vi "Connect FSV.vi"(8 "error in (no error)":errorcluster caption="에러 입력(에러 없음)", 10 "VISA resource name":refnum<visa-resource-name>, 11 "Instrument Manager 입력":refnum<class "Instrument Manager.lvclass">) -> (0 "error out":errorcluster caption="에러 출력", 3 "Instrument Manager 출력":refnum<class "Instrument Manager.lvclass">)   [LabVIEW 2023, in "Instrument Manager.lvclass"]
uses:
  Instrument Manager.lvclass
  Instrument Manager.lvclass/Instrument Manager.ctl
  Module/Spectrum Analyzer/Class/FSV-40N/FSV-40N.lvclass
  C:/Users/HCT-3320/Documents/Instrument Manger/Module/Spectrum Analyzer/Class/FSV-40N/FSV-40N.lvclass
  C:/Users/HCT-3320/Documents/Instrument Manger/Module/Spectrum Analyzer/Interface_Spectrum/Interface_Spectrum.lvclass
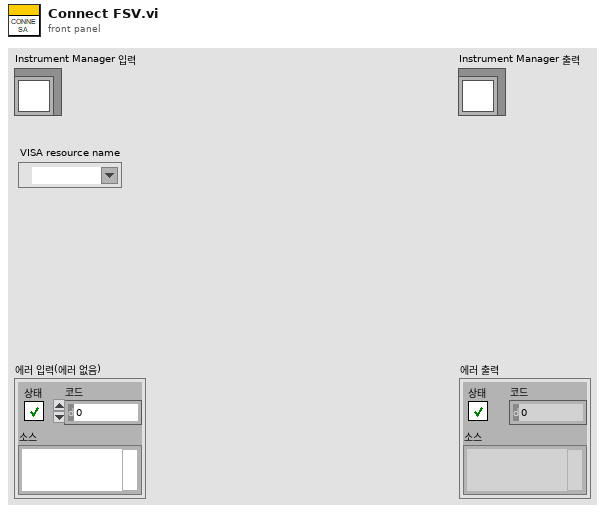
[diagram p1: front panel]
types:
  T1 = cluster{"Anritsu Call Box":refnum<class "Anritsu Call Box.lvclass">, "Spectrum Analyzer":refnum<class "Interface_Spectrum.lvclass">, "RF Switch Box":refnum<class "RF Filter Box.lvclass">, "Turn Table":refnum<class "Interface - Turn Table.lvclass">, "Mast":refnum<class "Interface - Mast.lvclass">, "3D Controller":refnum<class "Interface_3D Controller.lvclass">}
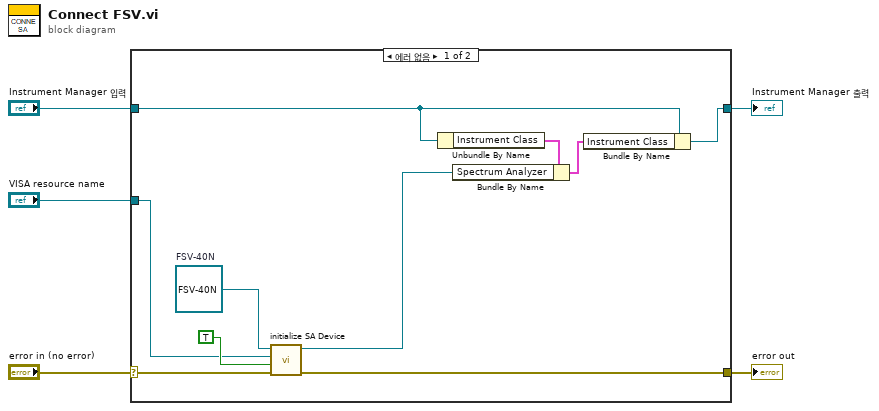
[diagram p0: block diagram]
diagram:
  n1 = case shown="에러 없음" "error in (no error)" {
    selector: "error in (no error)" -> [w14 w17]
    tunnel: [w6 w17] -> w4
    tunnel: [w12 w16] -> w2
    tunnel: "Instrument Manager 입력" -> [w13 w16]
    tunnel: "VISA resource name" -> [w7 _]
    frame No Error {
      w15 = refnum<class "FSV-40N.lvclass"> refnum  # FSV-40N
      n2 = call-dynamic "initialize SA Device.vi"("error in (no error)"=w14, "S.A Reset?"=TRUE, "VISA resource name"=w7, "FSV-40N in"=w15) -> ("error out"=w6:errorcluster, "FSV-40N out"=w9:refnum<class "FSV-40N.lvclass">)  [unwired: 6 in]
      n3 = Unbundle By Name(w13) -> ("Instrument Class"=w11:T1)
      n4 = Bundle By Name(cluster=w11, "Spectrum Analyzer"=w9) -> (w10:T1)
      n5 = Bundle By Name(cluster=w13, "Instrument Class"=w10) -> (w12:refnum<class "Instrument Manager.lvclass">)
    }
    frame Error {
    }
  }
  "error out" <- w4
  "Instrument Manager 출력" <- w2
